vi "set FCC Part15c U-NII-1 Standard BE mode.vi"(8 "error in (no error)":errorcluster, 11 "Band Edge in":refnum<class "Band Edge.lvclass">) -> (0 "error out":errorcluster, 3 "Band Edge out":refnum<class "Band Edge.lvclass">)   [LabVIEW 2023, in "Spectrum Analyzer.lvlib" / "Band Edge.lvclass"]
uses:
  Band Edge.lvclass
  Band Edge.lvclass/Band Edge.ctl
  Interface_Spectrum/Interface_Spectrum.lvclass
  TYPE DEFINITION/TYPE RBW and VBW Select.ctl
  Spectrum Analyzer.lvlib
  TYPE DEFINITION/TYPE Reference Level and Atten Param.ctl
  TYPE DEFINITION/TYPE Y-axis Unit.ctl
  TYPE DEFINITION/TYPE Sweep Type Select.ctl
  TYPE DEFINITION/TYPE Marker Auto Select.ctl
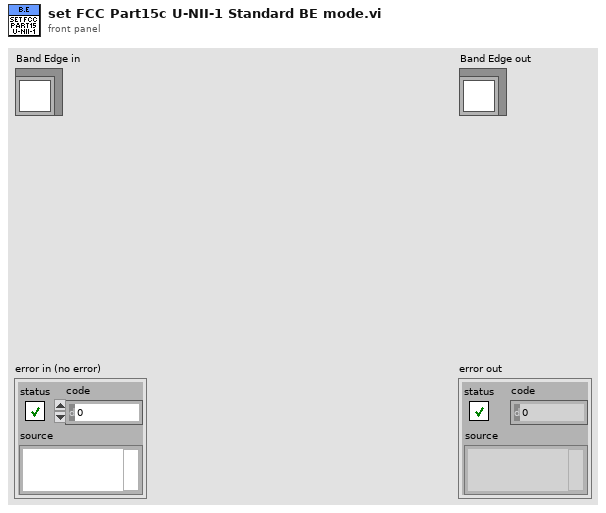
[diagram p1: front panel]
types:
  T1 = typedef "Spectrum Analyzer.lvlib/TYPE Marker Auto Select.ctl" = enum16{"Max Search Auto", "Min Search Auto"}
  T2 = typedef "Spectrum Analyzer.lvlib/TYPE Sweep Type Select.ctl" = enum16{"Auto", "Sweep", "FFT"}
  T3 = typedef "Spectrum Analyzer.lvlib/TYPE Y-axis Unit.ctl" = enum16{"dBm", "dBmV", "dBuV", "dBpW", "Volt", "Ampere", "Watt"}
  T4 = typedef "Spectrum Analyzer.lvlib/TYPE Reference Level and Atten Param.ctl" = cluster{"Reference Level":dbl, "Atten":i32, "Atten Auto?":bool, "Reference Level Offset":dbl}
  T5 = typedef "Spectrum Analyzer.lvlib/TYPE RBW and VBW Select.ctl" = enum16{"Res BW", "Video BW"}
  T6 = typedef "Spectrum Analyzer.lvlib/TYPE Spectrum Window Select.ctl" = enum16{"Spectrum 1", "Spectrum 2", "Spectrum 3", "Spectrum 4"}
  T7 = typedef "Spectrum Analyzer.lvlib/TYPE Start and Stop Frequency.ctl" = cluster{"Start":dbl, "Stop":dbl}
  T8 = typedef "Spectrum Analyzer.lvlib/TYPE Display Trace Mode Select.ctl" = enum16{"Clear Write", "Max Hold", "Min Hold", "Average", "View"}
  T9 = typedef "Spectrum Analyzer.lvlib/TYPE Detect Mode Select.ctl" = enum16{"Det Auto (Normal)", "Auto Peak", "Positive Peak", "Negative Peak", "Sample", "RMS", "Average", "Quasipeak", "CISPR Average", "RMS Average"}
  T10 = typedef "Spectrum Analyzer.lvlib/TYPE Marker Search Limit Set.ctl" = cluster{"Left Limit":dbl, "Right Limit":dbl, "Activate?":bool}
  T11 = typedef "Spectrum Analyzer.lvlib/TYPE Frequency Line Param.ctl" = cluster{"Line 1":dbl, "Line 2":dbl, "Activate Line1?":bool, "Activate Line2?":bool}
  T12 = typedef "Spectrum Analyzer.lvlib/TYPE Marker Value.ctl" = cluster{"X-axis":dbl, "Y-axis":dbl}
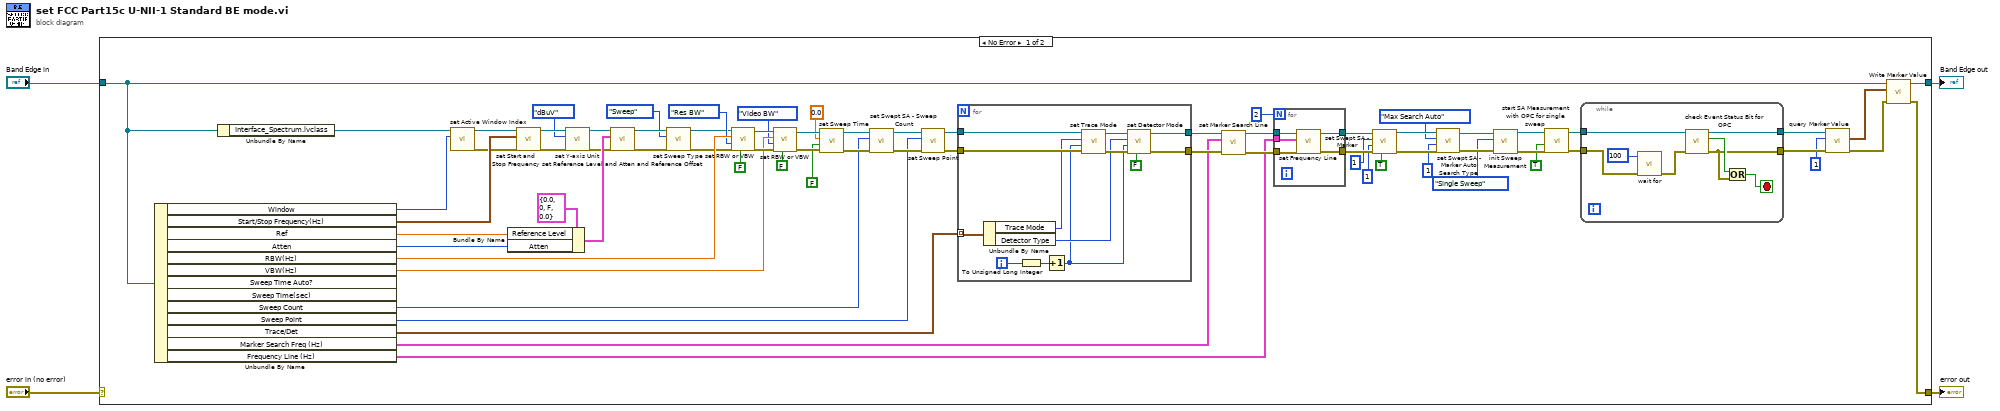
[diagram p0: block diagram]
diagram:
  n1 = case shown="No Error" "error in (no error)" {
    selector: "error in (no error)" -> [_ w104]
    tunnel: [w8 w104] -> w3
    tunnel: [w11 w103] -> w1
    tunnel: "Band Edge in" -> [w7 w103]
    frame No Error {
      n2 = Unbundle By Name(w7) -> ("Window"=w51:T6, "Start/Stop Frequency(Hz)"=w76:T7, "Ref"=w55:dbl, "Atten"=w54:i32, "RBW(Hz)"=w75:dbl, "VBW(Hz)"=w69:dbl, "Sweep Count"=w63:u32, "Sweep Point"=w60:u32, "Trace/Det"=w57:cluster{"Trace Mode":T8, "Detector Type":T9}[], "Marker Search Freq (Hz)"=w36:T10, "Frequency Line (Hz)"=w33:T11)  [unwired: 2 out]
      n3 = Unbundle By Name(w7) -> ("Interface_Spectrum.lvclass"=w52:refnum<class "Interface_Spectrum.lvclass">)
      n4 = call-dynamic "set Active Window Index.vi"("Window"=w51, "Interface_Spectrum in"=w52) -> ("error out"=w49:errorcluster, "Interface_Spectrum out"=w50:refnum<class "Interface_Spectrum.lvclass">)  [unwired: 8 in]
      n5 = Bundle By Name(cluster=T4 {"Reference Level"=0.0, "Atten"=0, "Atten Auto?"=FALSE, "Reference Level Offset"=0.0} ("Ref and Atten"), "Reference Level"=w55, "Atten"=w54) -> (w53:T4)
      n6 = call-dynamic "set Start and Stop Frequency.vi"("error in (no error)"=w49, "Start/Stop Frequency(Hz)"=w76, "Interface_Spectrum in"=w50) -> ("error out"=w47:errorcluster, "Interface_Spectrum out"=w48:refnum<class "Interface_Spectrum.lvclass">)  [unwired: 7 in]
      n7 = call-dynamic "set Y-axis Unit.vi"("error in (no error)"=w47, "Y-axis Unit"=TYPE_Y-axis_Unit."dBuV", "Interface_Spectrum in"=w48) -> ("error out"=w45:errorcluster, "Interface_Spectrum out"=w46:refnum<class "Interface_Spectrum.lvclass">)  [unwired: 7 in]
      n8 = call-dynamic "set Reference Level and Atten and Reference Offset.vi"("error in (no error)"=w45, "Reference Level, Atten, Reference Offset"=w53, "Interface_Spectrum in"=w46) -> ("error out"=w42:errorcluster, "Interface_Spectrum out"=w43:refnum<class "Interface_Spectrum.lvclass">)  [unwired: 7 in]
      n9 = call-dynamic "set Sweep Type.vi"("error in (no error)"=w42, "Sweep Mode"=TYPE_Sweep_Type_Select."Sweep", "Interface_Spectrum in"=w43) -> ("error out"=w40:errorcluster, "Interface_Spectrum out"=w41:refnum<class "Interface_Spectrum.lvclass">)  [unwired: 7 in]
      n10 = call-dynamic "set RBW or VBW.vi"("BW Auto?"=FALSE, "error in (no error)"=w40, "BW Type"=TYPE_RBW_and_VBW_Select."Res BW", "BW Value (Hz)"=w75, "Interface_Spectrum in"=w41) -> ("error out"=w72:errorcluster, "Interface_Spectrum out"=w73:refnum<class "Interface_Spectrum.lvclass">)  [unwired: 5 in]
      n11 = call-dynamic "set RBW or VBW.vi"("BW Auto?"=FALSE, "error in (no error)"=w72, "BW Type"=TYPE_RBW_and_VBW_Select."Video BW", "BW Value (Hz)"=w69, "Interface_Spectrum in"=w73) -> ("error out"=w66:errorcluster, "Interface_Spectrum out"=w67:refnum<class "Interface_Spectrum.lvclass">)  [unwired: 5 in]
      n12 = call-dynamic "set Sweep Time.vi"("error in (no error)"=w66, "Sweep Time Auto?"=FALSE, "Sweep Time(sec)"=0.0, "Interface_Spectrum in"=w67) -> ("error out"=w64:errorcluster, "Interface_Spectrum out"=w65:refnum<class "Interface_Spectrum.lvclass">)  [unwired: 6 in]
      n13 = call-dynamic "set Swept SA - Sweep Count.vi"("error in (no error)"=w64, "Sweep Count"=w63, "Interface_Spectrum in"=w65) -> ("error out"=w61:errorcluster, "Interface_Spectrum out"=w62:refnum<class "Interface_Spectrum.lvclass">)  [unwired: 7 in]
      n14 = call-dynamic "set Sweep Point.vi"("error in (no error)"=w61, "Sweep Point"=w60, "Interface_Spectrum in"=w62) -> ("error out"=w58:errorcluster, "Interface_Spectrum out"=w59:refnum<class "Interface_Spectrum.lvclass">)  [unwired: 7 in]
      n15 = for {
        tunnel: w59 -> [w102]
        tunnel: w58 -> [w101]
        tunnel: w57 -> [w97] mode=indexing
        tunnel: [w91] -> w38
        tunnel: [w90] -> w37
        i -> [w94]
        n16 = Unbundle By Name(w97) -> ("Trace Mode"=w96:T8, "Detector Type"=w95:T9)
        n17 = To Unsigned Long Integer(number=w94) -> (unsigned 32bit integer=w92:u32)
        n18 = Increment(x=w92) -> (x+1=w93:u32)
        n19 = call-dynamic "set Trace Mode.vi"("error in (no error)"=w101, "Trace Index"=w93, "Trace Mode"=w96, "Interface_Spectrum in"=w102) -> ("error out"=w99:errorcluster, "Interface_Spectrum out"=w100:refnum<class "Interface_Spectrum.lvclass">)  [unwired: 6 in]
        n20 = call-dynamic "set Detector Mode.vi"("Detect Auto?"=FALSE, "error in (no error)"=w99, "Trace Index"=w93, "Detector Type"=w95, "Interface_Spectrum in"=w100) -> ("error out"=w90:errorcluster, "Interface_Spectrum out"=w91:refnum<class "Interface_Spectrum.lvclass">)  [unwired: 5 in]
      }
      n21 = call-dynamic "set Marker Search Line.vi"("error in (no error)"=w37, "Marker Search Freq (Hz)"=w36, "Interface_Spectrum in"=w38) -> ("error out"=w34:errorcluster, "Interface_Spectrum out"=w35:refnum<class "Interface_Spectrum.lvclass">)  [unwired: 7 in]
      n22 = for {
        N: 2 -> [_]
        tunnel: w35 -> [w89]
        tunnel: w34 -> [w88]
        tunnel: w33 -> [w87]
        tunnel: [w86] -> w31
        tunnel: [w85] -> w30
        n23 = call-dynamic "set Frequency Line.vi"("error in (no error)"=w88, "Frequency Line (Hz)"=w87, "Interface_Spectrum in"=w89) -> ("error out"=w85:errorcluster, "Interface_Spectrum out"=w86:refnum<class "Interface_Spectrum.lvclass">)  [unwired: 7 in]
      }
      n24 = call-dynamic "set Swept SA - Marker.vi"("On?"=TRUE, "error in (no error)"=w30, "trace"=1, "Index"=1, "Interface_Spectrum in"=w31) -> ("error out"=w25:errorcluster, "Interface_Spectrum out"=w26:refnum<class "Interface_Spectrum.lvclass">)  [unwired: 5 in]
      n25 = call-dynamic "set Swept SA - Marker Auto Search Type.vi"("error in (no error)"=w25, "Index"=1, "Marker Auto Type"=TYPE_Marker_Auto_Select."Max Search Auto", "Interface_Spectrum in"=w26) -> ("error out"=w21:errorcluster, "Interface_Spectrum out"=w22:refnum<class "Interface_Spectrum.lvclass">)  [unwired: 6 in]
      n26 = call-dynamic "init Sweep Measurement.vi"("error in (no error)"=w21, "Sweep Measurement Mode"=enum16{"Single Sweep", "Continuous Sweep"}."Single Sweep", "Interface_Spectrum in"=w22) -> ("error out"=w18:errorcluster, "Interface_Spectrum out"=w19:refnum<class "Interface_Spectrum.lvclass">)  [unwired: 7 in]
      n27 = call-dynamic "start SA Measurement with OPC for single sweep.vi"("error in (no error)"=w18, "with OPC?"=TRUE ("Check OPC?"), "Interface_Spectrum in"=w19) -> ("error out"=w15:errorcluster, "Interface_Spectrum out"=w16:refnum<class "Interface_Spectrum.lvclass">)  [unwired: 7 in]
      n28 = while {
        tunnel: w16 -> [w84]
        tunnel: w15 -> [w83]
        tunnel: [w79] -> w14
        tunnel: [w77] -> w13
        stop <- w80 stop-if-true
        n29 = call "wait for.vi"("error in"=w83, "Wait Time (ms)"=100) -> ("error out"=w82:errorcluster)  [unwired: 9 in]
        n30 = call-dynamic "check Event Status Bit for OPC.vi"("error in (no error)"=w82, "Interface_Spectrum in"=w84) -> ("error out"=w79:errorcluster, "OPC Bit Changed?"=w81:bool, "Interface_Spectrum out"=w77:refnum<class "Interface_Spectrum.lvclass">)  [unwired: 7 in]
        n31 = Or(x=w81, y=w79) -> (x .or. y?=w80:bool)
      }
      n32 = call-dynamic "query Marker Value.vi"("error in (no error)"=w14, "Marker Index"=1, "Interface_Spectrum in"=w13) -> ("error out"=w9:errorcluster, "Marker Value"=w10:T12)  [unwired: 6 in, 1 out]
      n33 = call "Write Marker Value.vi"("error in (no error)"=w9, "Marker Value"=w10, "Band Edge in"=w7) -> ("error out"=w8:errorcluster, "Band Edge out"=w11:refnum<class "Band Edge.lvclass">)  [unwired: 7 in]
    }
    frame Error {
    }
  }
  "error out" <- w3
  "Band Edge out" <- w1
